vi "Sous_VI_RT_Lanceur.vi"(8 "Erreur_in":errorcluster caption="Erreur", 10 "cpt_in":i32, 11 "enum_in":T1) -> (0 "Erreur_out":errorcluster caption="Erreur", 1 "vi_fini":bool, 2 "cpt_out":i32, 3 "enum_out":T1, 5 "Détection de ligne":bool[](array[boolean]))   [LabVIEW 2018]
doc: "Lance des balles sur une cible"
uses:
  enum_RT_lanceur.ctl
  enum_moteur_lanceur.ctl
  enum_distributeur_lanceur.ctl
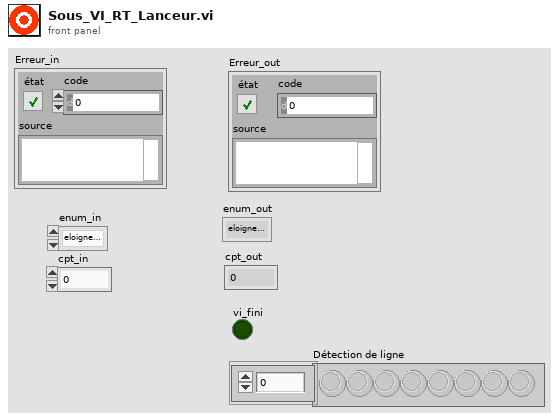
[diagram p1: front panel]
types:
  T1 = typedef "enum_RT_lanceur.ctl" = enum16{"eloignement", "arret_robot", "moteur_lanceur", "distributeur", "arret_distributeur_lanceur"}
  T2 = typedef "enum_moteur_lanceur.ctl" = enum16{"distance", "sans_distance", "desactive"}
  T3 = typedef "enum_distributeur_lanceur.ctl" = enum16{"Arret", "Marche"}
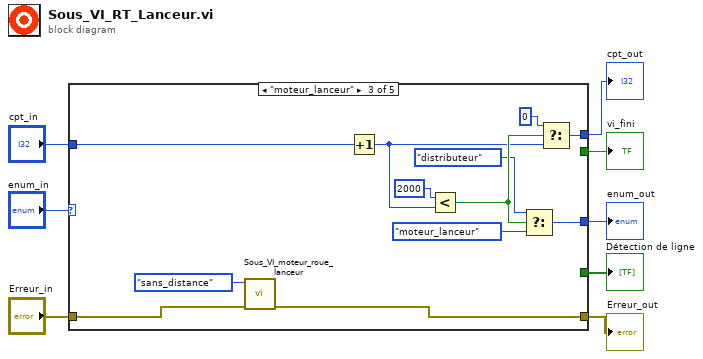
[diagram p0: block diagram]
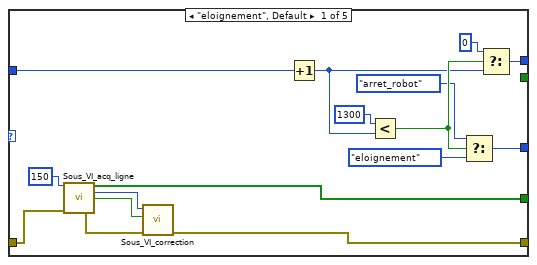
[diagram p2: hidden frame]
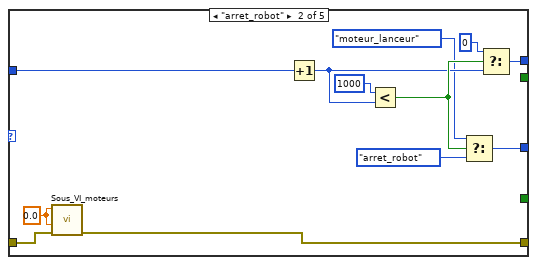
[diagram p3: hidden frame]
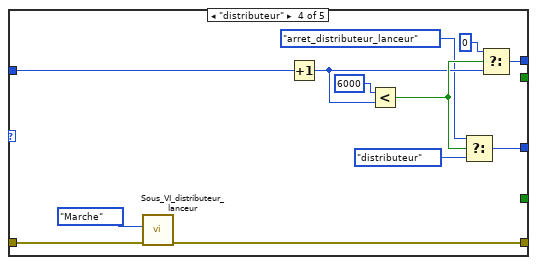
[diagram p4: hidden frame]
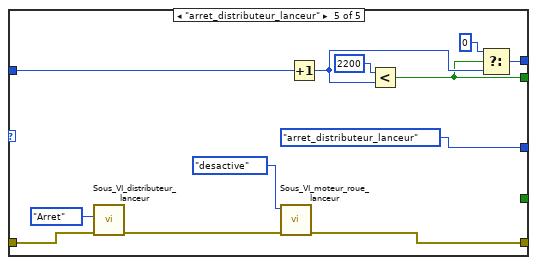
[diagram p5: hidden frame]
diagram:
  n1 = case shown="\"moteur_lanceur\"" "enum_in" {
    tunnel: "cpt_in" -> [w23 w34 w44 w56 w69]
    tunnel: [w17 w32 w43 w55 w68] -> w2
    tunnel: [w24 w35 w42 w54 enum_RT_lanceur."arret_distributeur_lanceur"] -> w3
    tunnel: "Erreur_in" -> [w13 w28 w40 w52 w64]
    tunnel: [w12 w27 w39 w51 w63] -> w7
    tunnel: [_ _ _ _ w62] -> w4
    tunnel: [w9 _ _ _ _] -> w1
    frame "eloignement", Default {
      n2 = call "Sous_VI_acq_ligne.vi"("Seuil"=150, "error in (no error)"=w13) -> ("x > y ?"=w9:bool[], "Décalage"=w18:u32, "G/D ?"=w20:bool, "error out"=w21:errorcluster)  [unwired: 8 in, 2 out]
      n3 = call "Sous_VI_correction.vi"("error in (no error)"=w21, "G/D ?"=w20, "Décalage"=w18) -> ("error out"=w12:errorcluster)  [unwired: 8 in]
      n4 = Increment(x=w23) -> (x+1=w15:i32)
      n5 = Less?(x=1300, y=w15) -> (x < y?=w16:bool)
      n6 = Select(t=enum_RT_lanceur."arret_robot", s=w16, f=enum_RT_lanceur."eloignement") -> (s? t:f=w24:T1)
      n7 = Select(t=0 ("cas vrai"), s=w16, f=w15) -> (s? t:f=w17:i32)
    }
    frame "arret_robot" {
      w33 = 0.0 ("Moteur Gauche")
      n8 = call "Sous_VI_moteurs.vi"("error in (no error)"=w28, "Moteur Droit"=w33, "Moteur Gauche"=w33) -> ("error out"=w27:errorcluster)  [unwired: 8 in]
      n9 = Increment(x=w34) -> (x+1=w30:i32)
      n10 = Less?(x=1000, y=w30) -> (x < y?=w31:bool)
      n11 = Select(t=enum_RT_lanceur."moteur_lanceur", s=w31, f=enum_RT_lanceur."arret_robot") -> (s? t:f=w35:T1)
      n12 = Select(t=0 ("cas vrai"), s=w31, f=w30) -> (s? t:f=w32:i32)
    }
    frame "moteur_lanceur" {
      n13 = call "Sous_VI_moteur_roue_lanceur.vi"("error in (no error)"=w40, "Mode"=enum_moteur_lanceur."sans_distance") -> ("error out"=w39:errorcluster)  [unwired: 9 in]
      n14 = Increment(x=w44) -> (x+1=w46:i32)
      n15 = Less?(x=2000, y=w46) -> (x < y?=w47:bool)
      n16 = Select(t=enum_RT_lanceur."distributeur", s=w47, f=enum_RT_lanceur."moteur_lanceur") -> (s? t:f=w42:T1)
      n17 = Select(t=0 ("cas vrai"), s=w47, f=w46) -> (s? t:f=w43:i32)
    }
    frame "distributeur" {
      n18 = call "Sous_VI_distributeur_lanceur.vi"("error in (no error)"=w52, "Enum"=enum_distributeur_lanceur."Marche") -> ("error out"=w51:errorcluster)  [unwired: 9 in]
      n19 = Increment(x=w56) -> (x+1=w58:i32)
      n20 = Less?(x=6000, y=w58) -> (x < y?=w59:bool)
      n21 = Select(t=enum_RT_lanceur."arret_distributeur_lanceur", s=w59, f=enum_RT_lanceur."distributeur") -> (s? t:f=w54:T1)
      n22 = Select(t=0 ("cas vrai"), s=w59, f=w58) -> (s? t:f=w55:i32)
    }
    frame "arret_distributeur_lanceur" {
      n23 = call "Sous_VI_distributeur_lanceur.vi"("error in (no error)"=w64, "Enum"=enum_distributeur_lanceur."Arret") -> ("error out"=w67:errorcluster)  [unwired: 9 in]
      n24 = call "Sous_VI_moteur_roue_lanceur.vi"("error in (no error)"=w67, "Mode"=enum_moteur_lanceur."desactive") -> ("error out"=w63:errorcluster)  [unwired: 9 in]
      n25 = Increment(x=w69) -> (x+1=w71:i32)
      n26 = Less?(x=2200, y=w71) -> (x < y?=w62:bool)
      n27 = Select(t=0 ("cas vrai"), s=w62, f=w71) -> (s? t:f=w68:i32)
    }
  }
  "Erreur_out" <- w7
  "vi_fini" <- w4
  "enum_out" <- w3
  "cpt_out" <- w2
  "Détection de ligne" <- w1
